vi "test_Remove Custom Device.vi"(8 "error in (no error)":errorcluster, 11 "TestCase in":refnum<class "Scan Engine Scripting API Custom Device Unit Tests.lvclass">) -> (0 "error out":errorcluster, 3 "TestCase out":refnum<class "Scan Engine Scripting API Custom Device Unit Tests.lvclass">)   [LabVIEW 2020, in "Scan Engine Scripting API Custom Device Unit Tests.lvclass"]
uses:
  Scan Engine Scripting API Custom Device Unit Tests.lvclass
  Shared/Type Defs/Main Settings.ctl
  Scan Engine Scripting API Custom Device Unit Tests.lvclass/Scan Engine Scripting API Custom Device Unit Tests.ctl
  <vilib>/addons/_JKI Toolkits/VI Tester/TestCase.llb/TestCase.lvclass
  Scripting/Scan Engine Scripting.lvlib
  Shared/SEECD Shared.lvlib
  C:/Program Files (x86)/National Instruments/LabVIEW 2020/vi.lib/addons/_JKI Toolkits/VI Tester/TestCase.llb/TestCase.lvclass
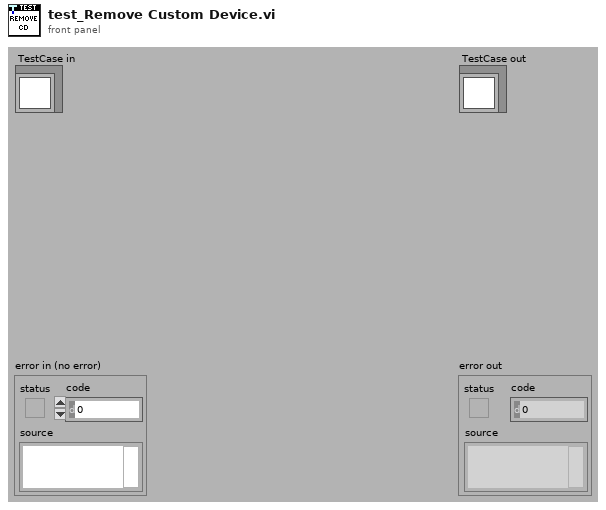
[diagram p1: front panel]
types:
  T1 = typedef "SEECD Shared.lvlib/Main Settings.ctl" = cluster{"sync to scan":bool, "scan engine decimation":u16, "delay after FPGA load (s)":u16}
  T2 = typedef "Custom Device API.lvlib/Custom Device Item Ref.ctl" = u64
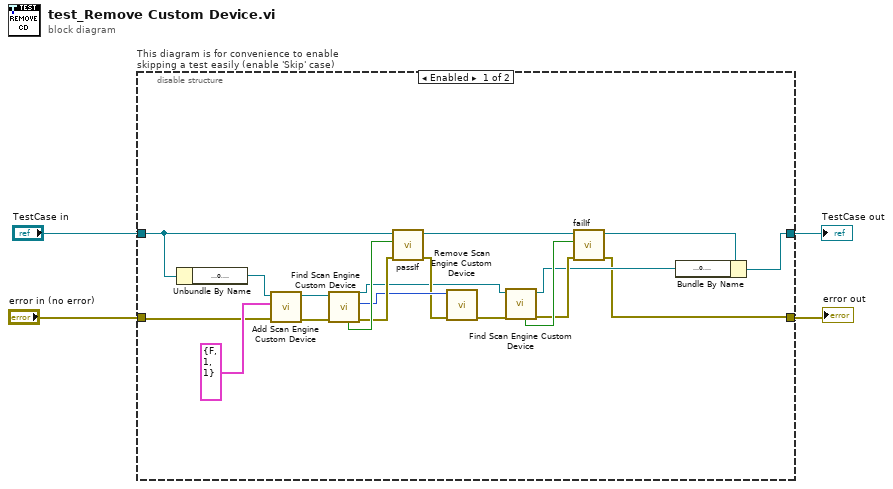
[diagram p0: block diagram]
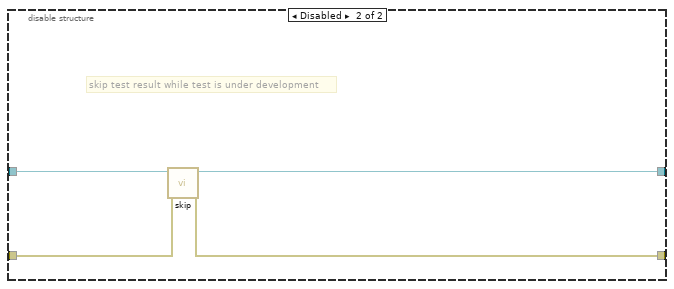
[diagram p2: hidden frame]
diagram:
  n1 = disable-structure "This diagram is for convenience to enable skipping a test easily (enable 'Skip' case)" shown="Enabled" {
    disable-tunnel: "TestCase in" -> [w11 w27]
    disable-tunnel: [w5 w25] -> w1
    disable-tunnel: [w6 w26] -> w3
    disable-tunnel: "error in (no error)" -> [w10 w24]
    frame Enabled {
      n2 = Unbundle By Name(w11) -> ("target ref"=w9:refnum<k24>)
      n3 = call "Add Scan Engine Custom Device.vi"("error in"=w10, "settings"=T1 {"sync to scan"=FALSE, "scan engine decimation"=1, "delay after FPGA load (s)"=1}, "target in"=w9) -> ("error out"=w22:errorcluster, "target out"=w21:refnum<k24>)  [unwired: 6 in, 1 out]
      n4 = call "Find Scan Engine Custom Device.vi"("error in"=w22, "target in"=w21) -> ("error out"=w19:errorcluster, "scan engine custom device ref"=w18:T2, "target out"=w15:refnum<k24>, "found"=w20:bool)  [unwired: 6 in]
      n5 = call-dynamic "passIf.vi"("error in (no error)"=w19, "pass"=w20, "TestCase in"=w11) -> ("error out"=w17:errorcluster, "TestCase out"=w13:refnum<class "Scan Engine Scripting API Custom Device Unit Tests.lvclass">)  [unwired: 7 in]
      n6 = call "Remove Scan Engine Custom Device.vi"("error in"=w17, "scan engine custom device ref in"=w18) -> ("error out"=w16:errorcluster)  [unwired: 9 in]
      n7 = call "Find Scan Engine Custom Device.vi"("error in"=w16, "target in"=w15) -> ("error out"=w12:errorcluster, "target out"=w7:refnum<k24>, "found"=w14:bool)  [unwired: 6 in, 1 out]
      n8 = call-dynamic "failIf.vi"("error in (no error)"=w12, "fail"=w14, "TestCase in"=w13) -> ("error out"=w6:errorcluster, "TestCase out"=w8:refnum<class "Scan Engine Scripting API Custom Device Unit Tests.lvclass">)  [unwired: 7 in]
      n9 = Bundle By Name(cluster=w8, "target ref"=w7) -> (w5:refnum<class "Scan Engine Scripting API Custom Device Unit Tests.lvclass">)
    }
    frame Disabled {
      # "skip test result while test is under development"
      n10 = call <vilib>:"skip.vi"("error in (no error)"=w24, "TestCase in"=w27) -> ("error out"=w26:errorcluster, "TestCase out"=w25:refnum<class "Scan Engine Scripting API Custom Device Unit Tests.lvclass">)  [unwired: 8 in]
    }
  }
  "error out" <- w3
  "TestCase out" <- w1
